vi "Close.vi"(8 "error in (no error)":errorcluster, 11 "bt_System in":refnum<class "bt_System.lvclass">) -> (0 "error out":errorcluster, 3 "bt_System out":refnum<class "bt_System.lvclass">)   [LabVIEW 2021, in "BT.lvlib" / "bt_System.lvclass"]
uses:
  bt_System.lvclass
  bt_System.lvclass/bt_System.ctl
  Support/Nodes/abs_Node/bt_Node.lvclass
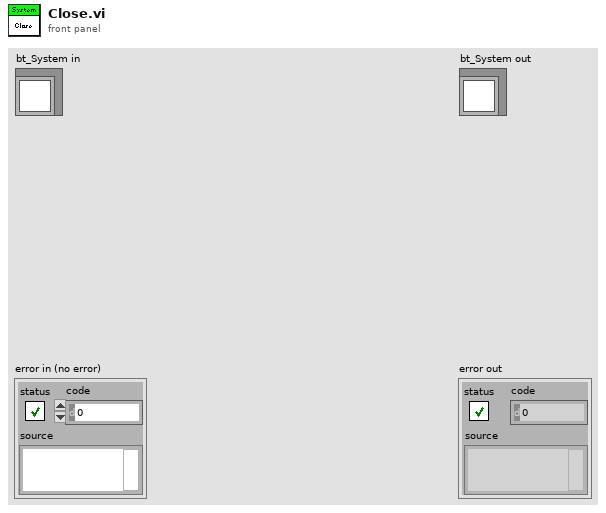
[diagram p1: front panel]
types:
  T1 = typedef "Rendezvous RefNum" = refnum<k1>
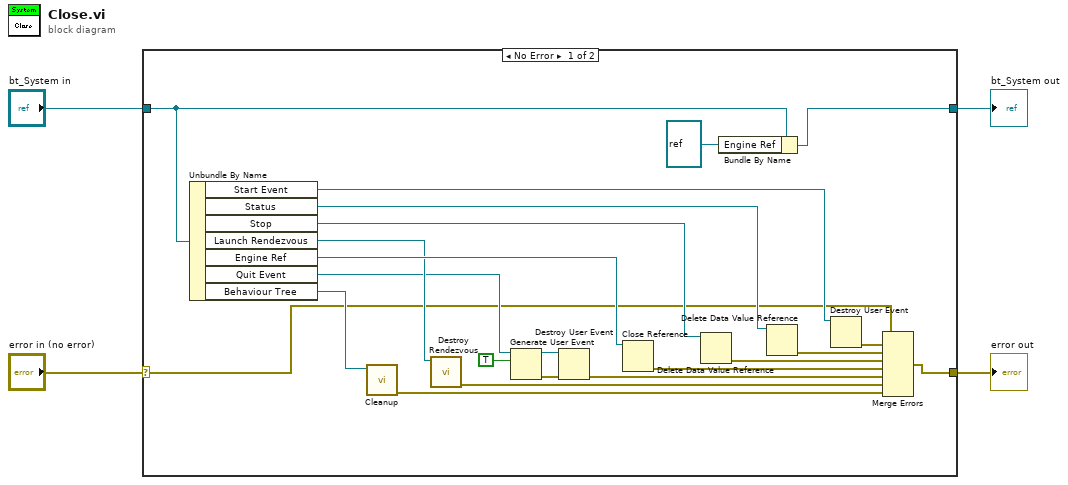
[diagram p0: block diagram]
diagram:
  n1 = case shown="No Error" "error in (no error)" {
    selector: "error in (no error)" -> [w5 w28]
    tunnel: [w12 w28] -> w3
    tunnel: [w25 w27] -> w1
    tunnel: "bt_System in" -> [w14 w27]
    frame No Error {
      n2 = Unbundle By Name(w14) -> ("Start Event"=w20:refnum<user-event>, "Status"=w21:refnum<data-value>, "Stop"=w22:refnum<data-value>, "Launch Rendezvous"=w23:T1, "Engine Ref"=w26:refnum<vi>, "Quit Event"=w16:refnum<user-event>, "Behaviour Tree"=w15:refnum<class "bt_Node.lvclass">)
      n3 = call-dynamic "Cleanup.vi"("Node in"=w15) -> ("error out"=w6:errorcluster)  [unwired: 9 in, 1 out]
      n4 = call <vilib>:"Destroy Rendezvous.vi"("rendezvous"=w23) -> ("error out"=w7:errorcluster)  [unwired: 5 in, 1 out]
      n5 = Generate User Event(user event=w16, event data cluster=TRUE ("event data")) -> (user event out=w18:refnum<user-event>, error out=w17:errorcluster)  [unwired: 2 in]
      n6 = Destroy User Event(user event=w18, error in=w17) -> (error out=w8:errorcluster)
      n7 = Close Reference(reference=w26) -> (error out=w9:errorcluster)  [unwired: 1 in]
      n8 = Delete Data Value Reference(data value reference=w22) -> (error out=w10:errorcluster)  [unwired: 1 in, 1 out]
      n9 = Bundle By Name(cluster=w14, "Engine Ref"=refnum<vi> refnum) -> (w25:refnum<class "bt_System.lvclass">)
      n10 = Delete Data Value Reference(data value reference=w21) -> (error out=w11:errorcluster)  [unwired: 1 in, 1 out]
      n11 = Destroy User Event(user event=w20) -> (error out=w13:errorcluster)  [unwired: 1 in]
      n12 = Merge Errors(w5, w13, w11, w10, w9, w8, w7, w6) -> (w12:errorcluster)
    }
    frame Error {
    }
  }
  "error out" <- w3
  "bt_System out" <- w1
